vi "Vacuum permissions.vi"(0 "attempt":u32, 1 "pos":u32, 2 "status":u32, 3 "site":u32, 4 "events":u32) -> (15 "alarms":u32)   [LabVIEW 2025]
doc: "Opening permission checks shared with the local Opta."
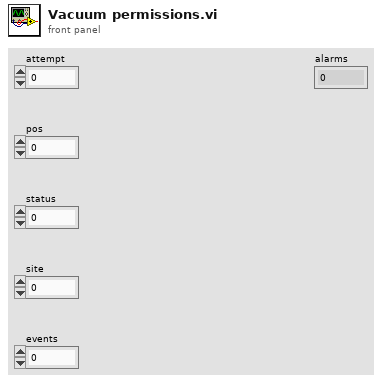
[diagram p1: front panel]
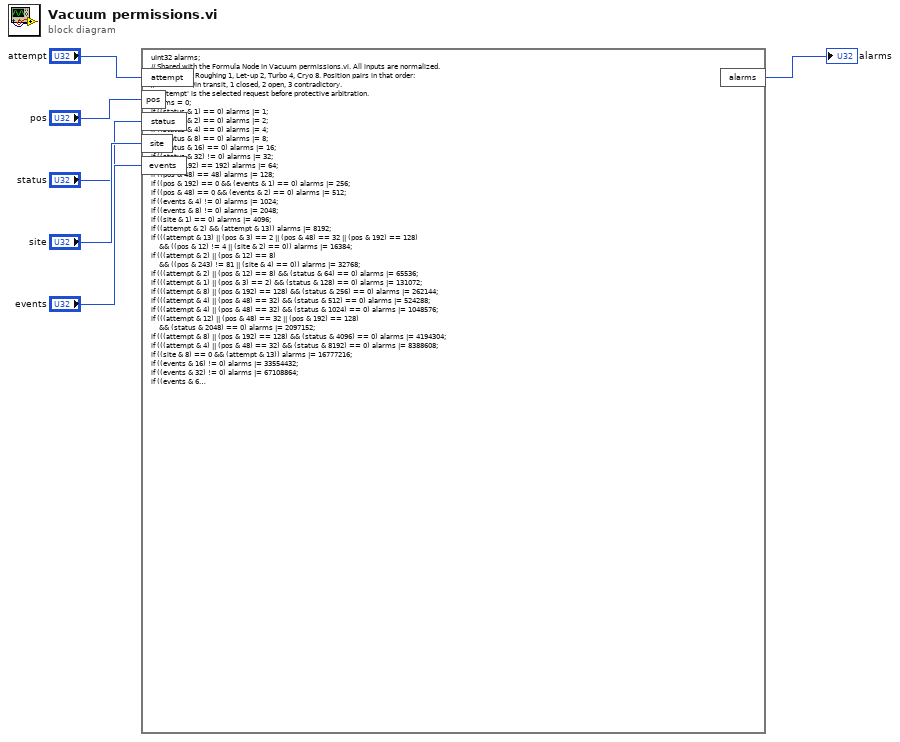
[diagram p0: block diagram]
diagram:
  n1 = formula code="uInt32 alarms;\n// Shared with the Formula Node in Vacuum permissions.vi. All inputs are normalized.\n// Valve bits: Roughing 1, Let-up 2, Turbo 4, Cryo 8. Position pairs in that order:\n// 0 unknown/in transit, 1 closed, 2 open, 3 contradictory.\n// 'attempt' is the selected request before protective arbitration.\nalarms = 0;\nif ((status & 1) == 0) alarms |= 1;\nif ((status & 2) == 0) alarms |= 2;\nif ((status & 4) == 0) alarms |= 4;\nif ((status & 8) == 0) alarms |= 8;\nif ((status & 16) == 0) alarms |= 16;\nif ((status & 32) != 0) alarms |= 32;\nif ((pos & 192) == 192) alarms |= 64;\nif ((pos & 48) == 48) alarms |= 128;\nif ((pos & 192) == 0 && (events & 1) == 0) alarms |= 256;\nif ((pos & 48) == 0 && (events & 2) == 0) alarms |= 512;\nif ((events & 4) != 0) alarms |= 1024;\nif ((events & 8) != 0) alarms |= 2048;\nif ((site & 1) == 0) alarms |= 4096;\nif ((attempt & 2) && (attempt & 13)) alarms |= 8192;\nif (((attempt & 13) || (pos & 3) == 2 || (pos & 48) == 32 || (pos & 192) == 128)\n    && ((pos & 12) != 4 || (site & 2) == 0)) alarms |= 16384;\nif (((attempt & 2) || (pos & 12) == 8)\n    && ((pos & 243) != 81 || (site & 4) == 0)) alarms |= 32768;\nif (((attempt & 2) || (pos & 12) == 8) && (status & 64) == 0) alarms |= 65536;\nif (((attempt & 1) || (pos & 3) == 2) && (status & 128) == 0) alarms |= 131072;\nif (((attempt & 8) || (pos & 192) == 128) && (status & 256) == 0) alarms |= 262144;\nif (((attempt & 4) || (pos & 48) == 32) && (status & 512) == 0) alarms |= 524288;\nif (((attempt & 4) || (pos & 48) == 32) && (status & 1024) == 0) alarms |= 1048576;\nif (((attempt & 12) || (pos & 48) == 32 || (pos & 192) == 128)\n    && (status & 2048) == 0) alarms |= 2097152;\nif (((attempt & 8) || (pos & 192) == 128) && (status & 4096) == 0) alarms |= 4194304;\nif (((attempt & 4) || (pos & 48) == 32) && (status & 8192) == 0) alarms |= 8388608;\nif ((site & 8) == 0 && (attempt & 13)) alarms |= 16777216;\nif ((events & 16) != 0) alarms |= 33554432;\nif ((events & 32) != 0) alarms |= 67108864;\nif ((events & 64) != 0) alarms |= 134217728;\nif (((attempt & 2) || (pos & 12) == 8) && (site & 16) == 0) alarms |= 268435456;\nif ((events & 128) != 0) alarms |= 536870912;\nif ((events & 256) != 0) alarms |= 1073741824;"("attempt"="attempt", "pos"="pos", "status"="status", "site"="site", "events"="events") -> ("alarms"=→"alarms":u32)
